vi "Flatten XNET CAN to pcap CAN.vi"(8 "error in (no error)":errorcluster, 10 "XNET CAN Data":T1[](array[typedef]) {"payload" format="%x"; "timestamp" format="%<%.7X\n%x>T"; "type" items=["CAN Data"=0, "CAN Remote"=1, "CAN Bus Error"=2, "CAN 2.0 Data"=8, "CAN FD Data"=16, "CAN FD+BRS Data"=24, "J1939 Data"=192, "Delay"=224, "Log Trigger"=225, "Start Trigger"=226]; "identifier" format="%x"}, 11 "XNET_CAN_RW in":refnum<class "XNET CAN RW.lvclass">) -> (0 "error out":errorcluster, 2 "pcap CAN DATA":u8[](array[numeric]), 5 "Number Filtered":u32)   [LabVIEW 2021, in "XNET CAN RW.lvclass"]
uses:
  XNET CAN RW.lvclass
  <vilib>/xnet/xnet.llb/XNET Frame CAN.ctl
  <vilib>/xnet/xnet.llb/XNET Frame Type CAN.ctl
  C:/Program Files/National Instruments/LabVIEW 2021/vi.lib/CIF Foundation/CIF CAN RW Core/CAN_RW_CORE.lvclass
  <vilib>/CIF Foundation/CIF CAN RW Core/CAN_RW_CORE.lvclass/CAN_RW_CORE.ctl
  <vilib>/CIF Foundation/CIF PCAP Parse and Build/pcap_Parse_Build_CIF.lvclass/pcap_Parse_Build_CIF.ctl
  <vilib>/CIF Foundation/CIF CAN RW Core/Accessors/Read CAN Interface Mode.vi
  <vilib>/CIF Foundation/CIF CAN RW Core/Accessors/Read pcap class.vi
  <vilib>/CIF Foundation/CIF Utilities/Time/System Time/LabVIEW Time to TAI Time.vi
  <vilib>/CIF Foundation/CIF PCAP Parse and Build/Build/SubVIs/Flatten Packet Header.vi
  <vilib>/CIF Foundation/CIF Utilities/DataTypes/Flatten Unflatten/Flatten U32.vi
  <vilib>/CIF Foundation/CIF PCAP Parse and Build/pcap_Parse_Build_CIF.lvclass
  <vilib>/CIF Foundation/CIF CAN RW Core/CAN_RW_CORE.lvclass
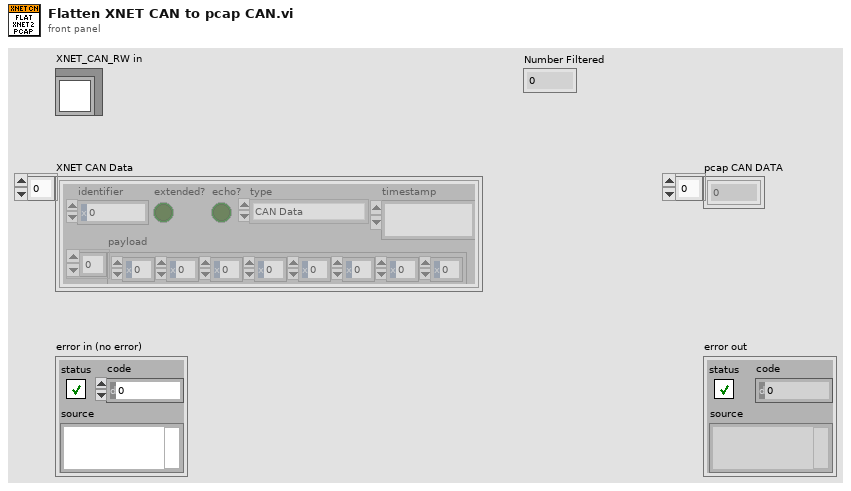
[diagram p1: front panel]
types:
  T1 = typedef "XNET Frame CAN.ctl" = cluster{"timestamp":timestamp, "payload":u8[], "identifier":u32, "type":T2, "extended?":bool, "echo?":bool}
  T2 = typedef "XNET Frame Type CAN.ctl" = u8
  T3 = typedef "CAN_RW_CORE.lvclass/CAN Interface Mode.ctl" = enum16{"Unknown", "CAN 2.0", "CAN FD", "CAN FD BRS"}
  T4 = typedef "pcap_Parse_Build_CIF.lvclass/Socket CAN Header.ctl" = cluster{"CANID and Flags":u32, "Payload Length":u8, "FD Flags":u8, "RSVD":u8, "Len8 DLC":u8}
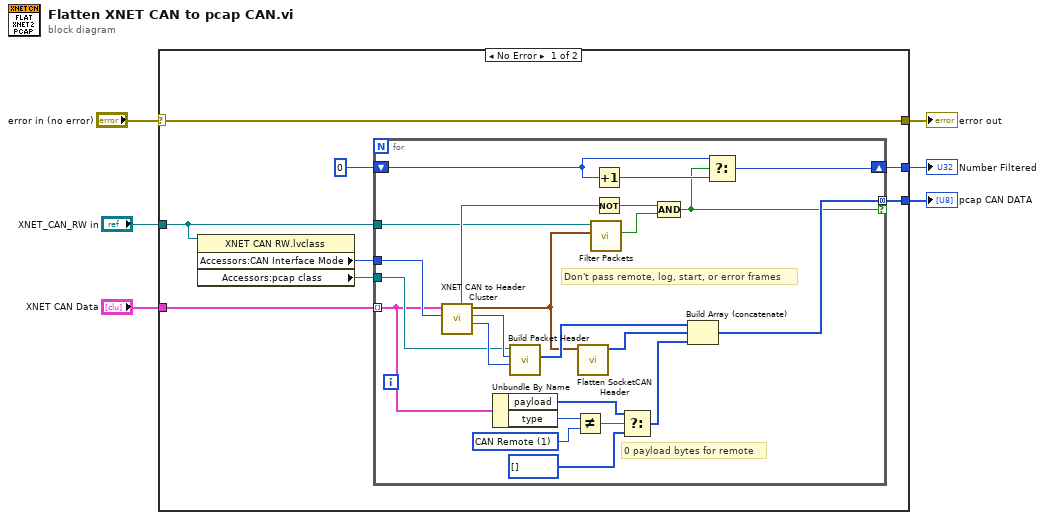
[diagram p0: block diagram]
diagram:
  n1 = case shown="No Error" "error in (no error)" {
    selector: "error in (no error)" -> [w9 w38]
    tunnel: [w14 _] -> w6
    tunnel: "XNET CAN Data" -> [w13 _]
    tunnel: "XNET_CAN_RW in" -> [w12 _]
    tunnel: [w9 w38] -> w2
    tunnel: [w7 _] -> w1
    frame No Error {
      n2 = property class="XNET CAN RW.lvclass"(reference=w12) -> ("Accessors:CAN Interface Mode"=w11:T3, "Accessors:pcap class"=w10:refnum<class "pcap_Parse_Build_CIF.lvclass">)  [unwired: 1 in, 2 out]
      n3 = for {
        tunnel: w13 -> [w31] mode=indexing
        tunnel: [w30] -> w14 mode=concatenating if=w15
        tunnel: w10 -> [w32]
        tunnel: w11 -> [w36]
        tunnel: w12 -> [w29]
        shift-right: [w16] -> w7
        shift-left: u32 0 -> [w17]
        w26 = T2 1 items=["CAN Data"=0, "CAN Remote"=1, "CAN Bus Error"=2, "CAN 2.0 Data"=8, "CAN FD Data"=16, "CAN FD+BRS Data"=24, "J1939 Data"=192, "Delay"=224, "Log Trigger"=225, "Start Trigger"=226] ("y")
        # "0 payload bytes for remote"
        # "Don't pass remote, log, start, or error frames"
        n4 = call "XNET CAN to Header Cluster.vi"("Interface Mode"=w36, "XNET CAN frame"=w31) -> ("Total Length"=w35:i32, "TAI Time (ns)"=w34:i64, "CAN Header out"=w21:T4, "Unsupported"=w37:bool)  [unwired: 6 in]
        n5 = Unbundle By Name(w31) -> ("payload"=w24:u8[], "type"=w27:T2)
        n6 = call <vilib>:"Build Packet Header.vi"("Length"=w35, "TAI Time (ns)"=w34, "pcap Parse and Build in"=w32) -> ("Flattened Data out"=w33:u8[])  [unwired: 7 in, 1 out]
        n7 = Not Equal?(x=w27, y=w26) -> (x != y?=w25:bool)
        n8 = call <vilib>:"Flatten SocketCAN Header.vi"("CAN Header in"=w21) -> ("Flattened Data out"=w20:u8[])  [unwired: 10 in]
        n9 = call <vilib>:"Filter Packets.vi"("CAN Header in"=w21, "CAN_RW_CORE"=w29) -> ("Valid"=w19:bool)  [unwired: 9 in]
        n10 = Increment(x=w17) -> (x+1=w18:u32)
        n11 = Not(x=w37) -> (.not. x?=w28:bool)
        n12 = Select(t=w24, s=w25, f=u8[] []) -> (s? t:f=w23:u8[])
        n13 = Compound Arithmetic op=AND(w28, w19) -> (w15:bool)
        n14 = Build Array (concatenate)(w33, w20, w23) -> (w30:u8[])
        n15 = Select(t=w17, s=w15, f=w18) -> (s? t:f=w16:u32)
      }
    }
    frame Error {
    }
  }
  "pcap CAN DATA" <- w6
  "error out" <- w2
  "Number Filtered" <- w1
